vi "TimerTestsForEXE.vi"(0 "EXE Path":path, 5 "Drona Tests PPL":path, 11 "error in":errorcluster) -> (15 "error out":errorcluster)   [LabVIEW 2016]
doc: "Run the Drona Tests in EXE"
uses:
  Drona.lvlib
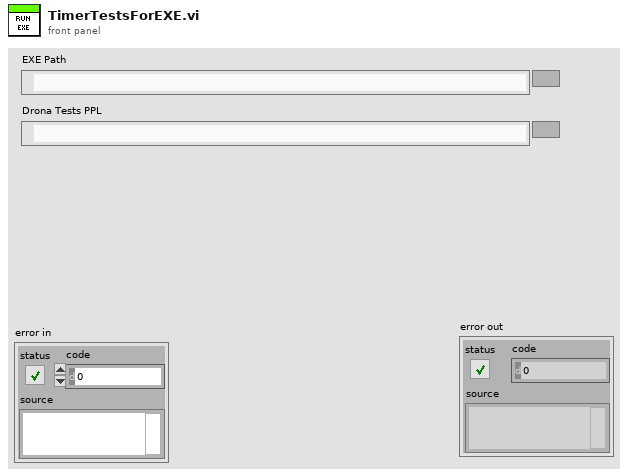
[diagram p1: front panel]
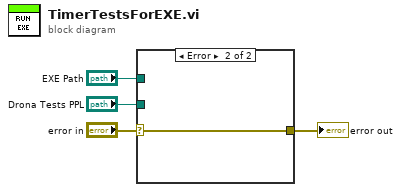
[diagram p0: block diagram]
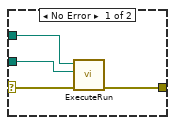
[diagram p2: hidden frame]
diagram:
  n1 = case shown="Error" "error in" {
    selector: "error in" -> [w8 w9]
    tunnel: "Drona Tests PPL" -> [w7 _]
    tunnel: "EXE Path" -> [w6 _]
    tunnel: [w5 w9] -> w1
    frame No Error {
      n2 = call "ExecuteRun.vi"("error in (no error)"=w8, "Drona Tests PPL"=w7, "EXE Path"=w6) -> ("error out"=w5:errorcluster)  [unwired: 8 in]
    }
    frame Error {
    }
  }
  "error out" <- w1
